vi "CNAL SQ array formation.vi"(11 "S New Info and MiN out":T2={"Sample Sequence"="GATGATGATGATGATGAT", "Right Read MIN"=6, "Filter P"=0, "STD Type"=enum."Region", "Base Table"=[], "Selection"=enum."10kHz", "noise MAX"=3, "Sample name"=""} {"Base Table"."Value 3" format="%.2g"}) -> (0 "Sample Sequence array":string[](array[string]), 2 "Sample name array":string[](array[string]), 3 "S array":T1(array[cluster]))   [LabVIEW 2018]
panel:
  in  "Recipe Name":string
  out "S array 2":T1(array[cluster])
  in  "Save":bool
  in  "load":bool
  in  "Delete":bool
  out "Total Try Sequence":i32
  in  "Insert":bool
  in  "Go_Next":bool
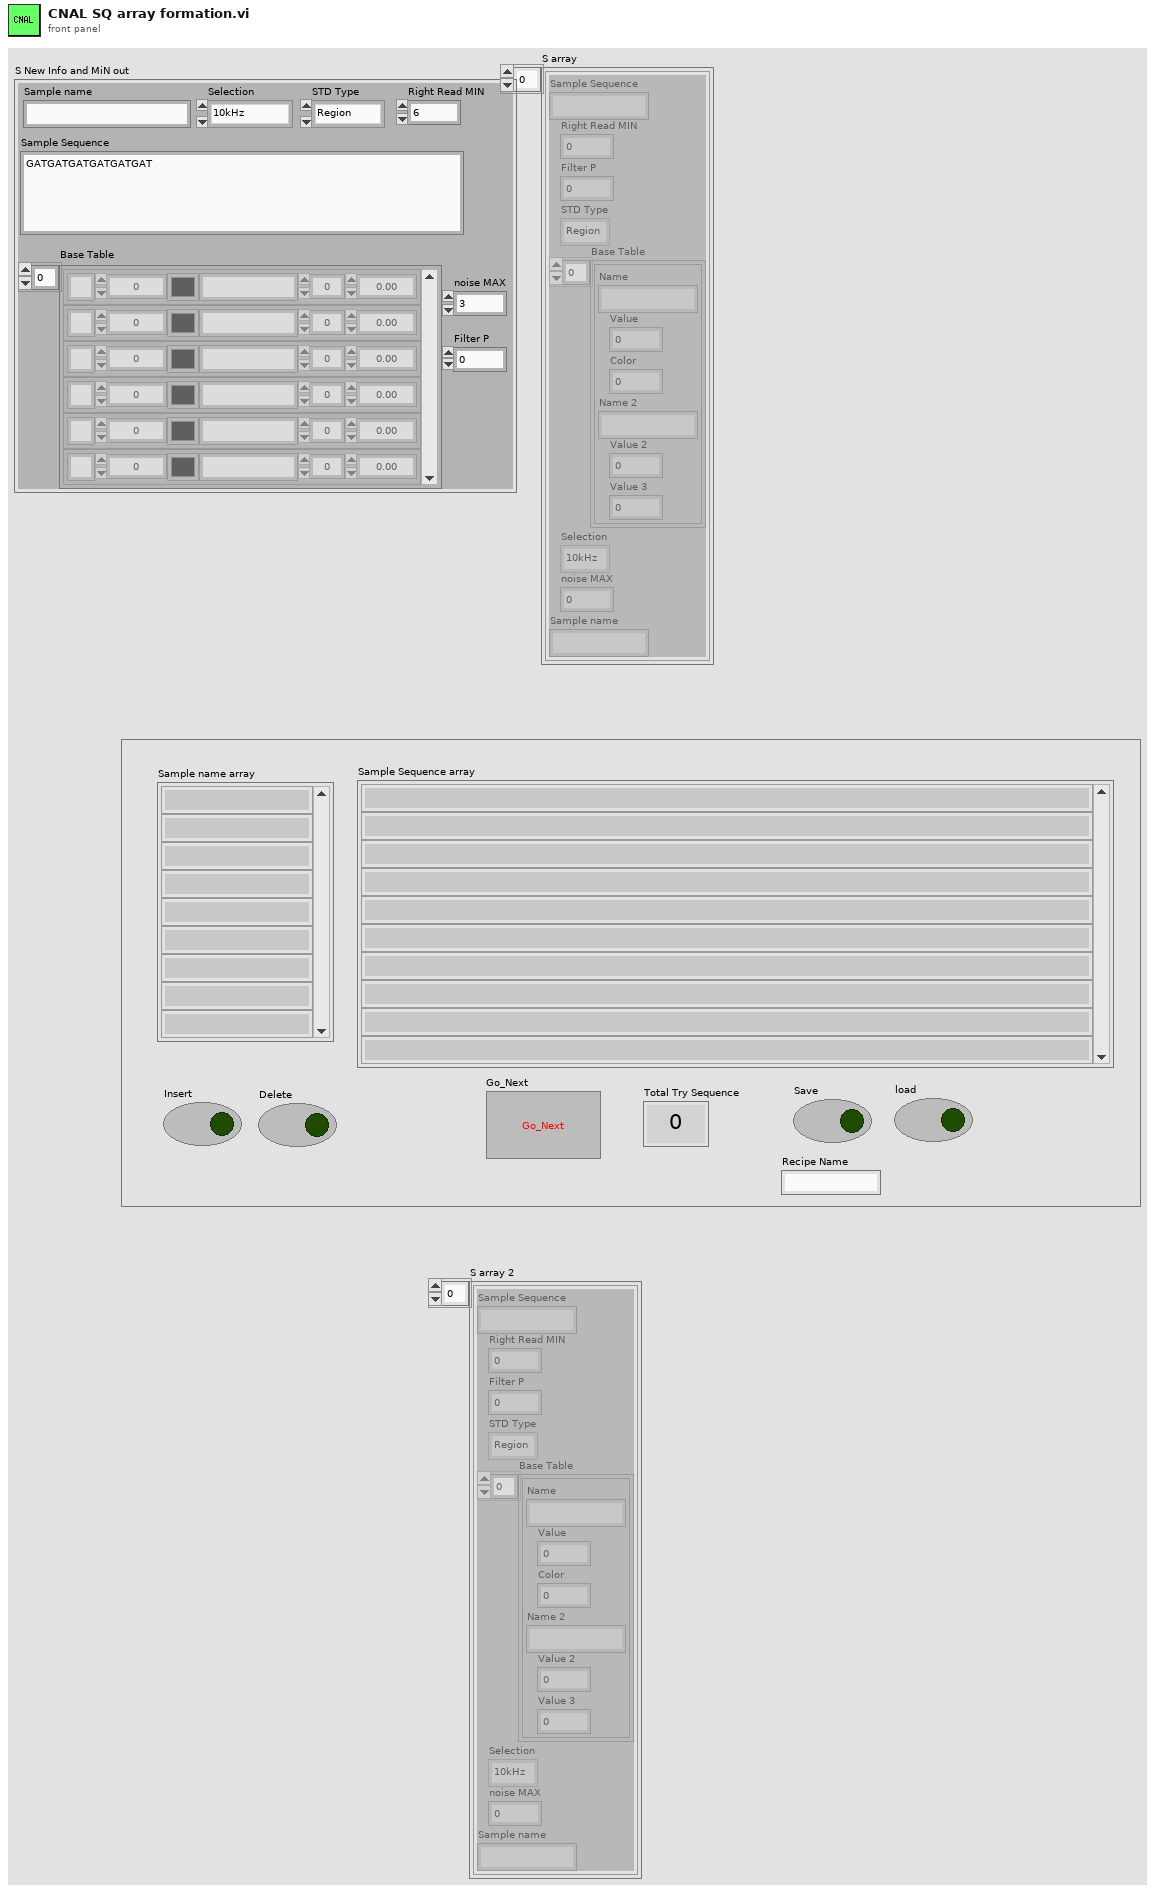
[diagram p1: front panel]
types:
  T1 = cluster{"Sample Sequence":string, "Right Read MIN":i32, "Filter P":i32, "STD Type":enum16{"Region", "Each", "Fixed"}, "Base Table":cluster{"Name":string, "Value":dbl, "Color":u32, "Name 2":string, "Value 2":dbl, "Value 3":dbl}[], "Selection":enum16{"10kHz", "100kHz"}, "noise MAX":i32, "Sample name":string}[]
  T2 = cluster{"Sample Sequence":string, "Right Read MIN":i32, "Filter P":i32, "STD Type":enum16{"Region", "Each", "Fixed"}, "Base Table":cluster{"Name":string, "Value":dbl, "Color":u32, "Name 2":string, "Value 2":dbl, "Value 3":dbl}[], "Selection":enum16{"10kHz", "100kHz"}, "noise MAX":i32, "Sample name":string}
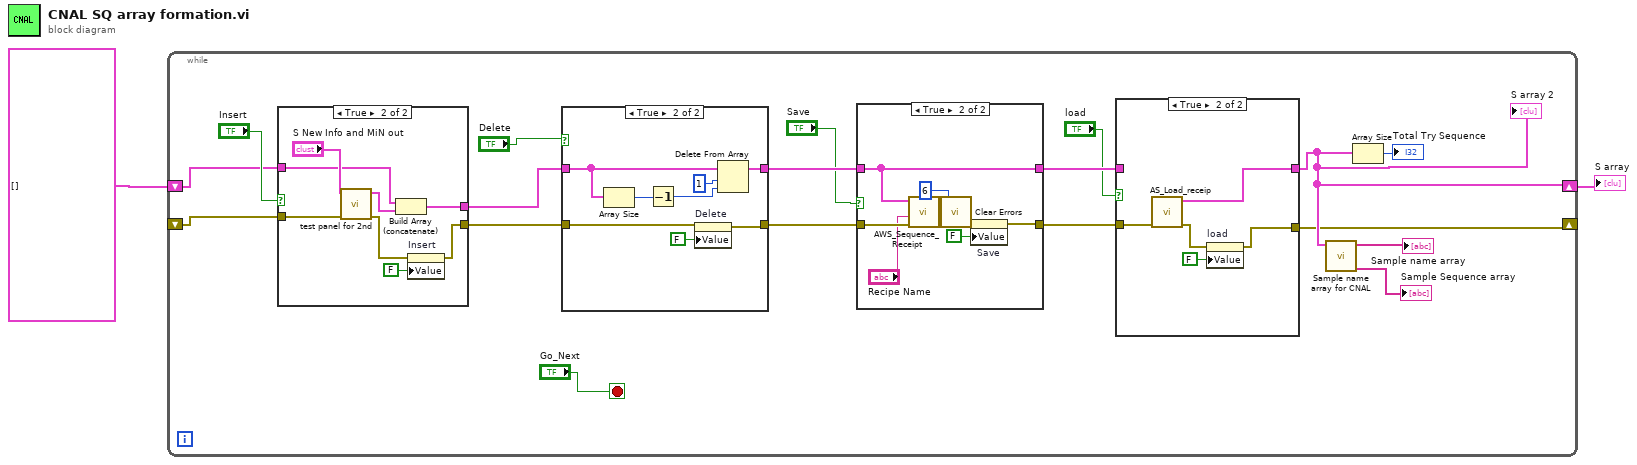
[diagram p0: block diagram]
diagram:
  n1 = while {
    shift-right: [w6] -> w2
    shift-left: T1 [] -> [w18]
    shift-right: [w4] -> _
    shift-left: _ -> [w17]
    stop <- "Go_Next" stop-if-true
    n2 = case shown="True" "Insert" {
      tunnel: [w49 w55] -> w12
      tunnel: w18 -> [w49 w54]
      tunnel: [w48 w51] -> w13
      tunnel: w17 -> [w48 w53]
      frame False {
      }
      frame True {
        n3 = call "test panel for 2nd.vi"("error in"=w53, "S New Info and MiN"="S New Info and MiN out") -> ("error out"=w52:errorcluster, "S New Info and MiN out"=w56:T2)  [unwired: 7 in, 1 out]
        n4 = Build Array (concatenate)(w54, w56) -> (w55:T1)
        n5 = property on="Insert" class="Bool (strict)"(error in=w52, "Value"=FALSE ("Boolean")) -> (error out=w51:errorcluster)  [unwired: 1 in, 1 out]
      }
    }
    n6 = case shown="True" "Delete" {
      tunnel: w13 -> [w39 w42]
      tunnel: [w39 w41] -> w9
      tunnel: w12 -> [w38 w43]
      tunnel: [w38 w44] -> w10
      frame False {
      }
      frame True {
        n7 = Array Size(array=w43) -> (size(s)=w46:i32)
        n8 = Decrement(x=w46) -> (x-1=w45:i32)
        n9 = property on="Delete" class="Bool (strict)"(error in=w42, "Value"=FALSE ("Delete")) -> (error out=w41:errorcluster)  [unwired: 1 in, 1 out]
        n10 = Delete From Array(array=w43, length=1 ("長さ"), index=w45) -> (array with subset deleted=w44:T1)  [unwired: 1 out]
      }
    }
    n11 = case shown="True" "Save" {
      tunnel: w10 -> [w29 w36]
      tunnel: [w29 w36] -> w7
      tunnel: w9 -> [w28 w37]
      tunnel: [w28 w33] -> w5
      frame False {
      }
      frame True {
        n12 = call "AWS_Sequence_Receipt.vi"("error in"=w37, "Save name"="Recipe Name", "S array"=w36) -> ("error out"=w34:errorcluster)  [unwired: 6 in, 2 out]
        n13 = call <vilib>:"Clear Errors.vi"("error in (no error)"=w34, "specific error code to clear (0: all)"=6) -> ("error out"=w31:errorcluster)  [unwired: 4 in, 1 out]
        n14 = property on="Save" class="Bool (strict)"(error in=w31, "Value"=FALSE ("Save")) -> (error out=w33:errorcluster)  [unwired: 1 in, 1 out]
      }
    }
    n15 = case shown="True" "load" {
      tunnel: w7 -> [w21 _]
      tunnel: [w21 w27] -> w6
      tunnel: w5 -> [w22 w26]
      tunnel: [w22 w24] -> w4
      frame False {
      }
      frame True {
        n16 = call "AS_Load_receip.vi"("error in"=w26) -> ("error out"=w25:errorcluster, "S array"=w27:T1)  [unwired: 9 in]
        n17 = property on="load" class="Bool (strict)"(error in=w25, "Value"=FALSE ("load")) -> (error out=w24:errorcluster)  [unwired: 1 in, 1 out]
      }
    }
    "S array 2" <- w6
    n18 = call "Sample name array for CNAL.vi"("S array"=w6) -> ("Sample Sequence array"=→"Sample Sequence array":string[], "Sample name array"=→"Sample name array":string[])  [unwired: 9 in]
    n19 = Array Size(array=w6) -> (size(s)=→"Total Try Sequence":i32)
  }
  "S array" <- w2
